vi "Triggered Tasks-Stop and Clear.vi"() -> (0 "error out":errorcluster)   [LabVIEW 2020]
uses:
  Globals/gl_Triggering globals.vi
  Global Variables/General Globals.vi
  Pockels/Globals/gl_Pockels control globals.vi
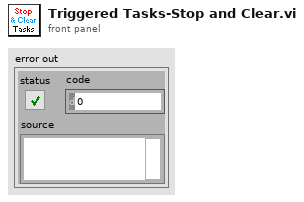
[diagram p1: front panel]
types:
  T1 = typedef "Triggered tasks cluster.ctl" = cluster{"DO task-Encoder trigger":refnum<k21>, "AO Task-Pockels modulation":refnum<k21>, "Counter Clock Task":refnum<k21>}
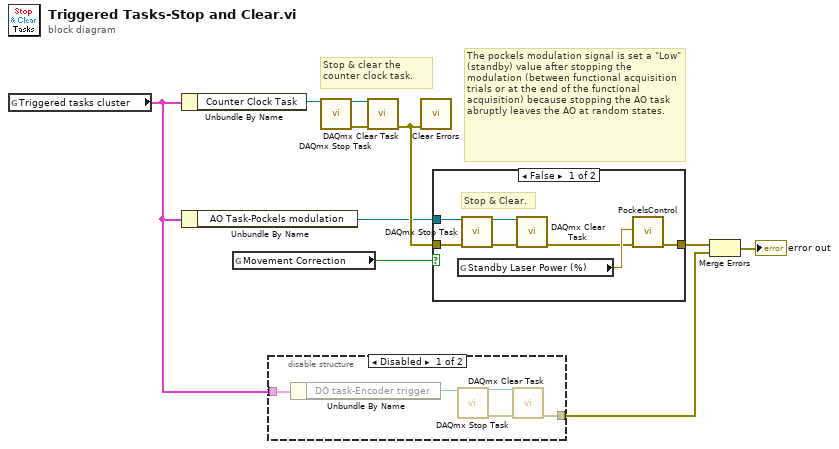
[diagram p0: block diagram]
diagram:
  # "The pockels modulation signal is set a \"Low\" (standby) value after stopping the modulation (between functional acquisition trials or at the end of the functional acquisition) because stopping the AO task abruptly leaves the AO at random states."
  # "Stop & clear the counter clock task."
  n1 = global read "gl_Triggering globals.vi" "Triggered tasks cluster"() -> (w5:T1)
  n2 = Unbundle By Name(w5) -> ("Counter Clock Task"=w7:refnum<k21>)
  n3 = Unbundle By Name(w5) -> ("AO Task-Pockels modulation"=w6:refnum<k21>)
  n4 = global read "General Globals.vi" "Movement Correction"() -> (w1:bool)
  n5 = disable-structure shown="Disabled" {
    disable-tunnel: [w15 _] -> w10
    disable-tunnel: w5 -> [w12 _]
    frame Disabled {
      n6 = Unbundle By Name(w12) -> ("DO task-Encoder trigger"=w13:refnum<k21>)
      n7 = call <vilib>:"DAQmx Stop Task.vi"("task/channels in"=w13) -> ("task out"=w11:refnum<k21>, "error out"=w14:errorcluster)  [unwired: 13 in]
      n8 = call <vilib>:"DAQmx Clear Task.vi"("task in"=w11, "error in"=w14) -> ("error out"=w15:errorcluster)  [unwired: 13 in]
    }
    frame Enabled {
    }
  }
  n9 = call <vilib>:"DAQmx Stop Task.vi"("task/channels in"=w7) -> ("task out"=w4:refnum<k21>, "error out"=w3:errorcluster)  [unwired: 13 in]
  n10 = call <vilib>:"DAQmx Clear Task.vi"("task in"=w4, "error in"=w3) -> ("error out"=w9:errorcluster)  [unwired: 13 in]
  n11 = call <vilib>:"Clear Errors.vi"("error in (no error)"=w9) -> ()  [unwired: 5 in, 2 out]
  n12 = case shown="False" w1 {
    tunnel: [w16 w23] -> w8
    tunnel: w6 -> [w20 _]
    tunnel: w9 -> [w19 w23]
    frame False {
      # "Stop & Clear."
      n13 = global read "gl_Pockels control globals.vi" "Standby Laser Power (%)"() -> (w18:dbl)
      n14 = call <vilib>:"DAQmx Stop Task.vi"("task/channels in"=w20, "error in"=w19) -> ("task out"=w22:refnum<k21>, "error out"=w21:errorcluster)  [unwired: 12 in]
      n15 = call <vilib>:"DAQmx Clear Task.vi"("task in"=w22, "error in"=w21) -> ("error out"=w17:errorcluster)  [unwired: 13 in]
      n16 = call "PockelsControl.vi"("Error In"=w17, "Laser Power (%)"=w18) -> ("Error Out"=w16:errorcluster)  [unwired: 9 in]
    }
    frame True {
    }
  }
  n17 = Merge Errors(w8, w10) -> (→"error out":errorcluster)
